vi "Measurement A.vi"(0 "Inputs":T1, 5 "Directory Path":path, 7 "First name":string, 9 "Last name":string, 11 "error in (no error)":errorcluster) -> (4 "Result":dbl, 6 "file or folder exists?":bool, 8 "Full name":string, 10 "dup path":path, 15 "error out":errorcluster)   [LabVIEW 2021]
uses:
  controls/Measurement Inputs.ctl
  controls/Offset value.ctl
  Reusables/controls/Username.ctl
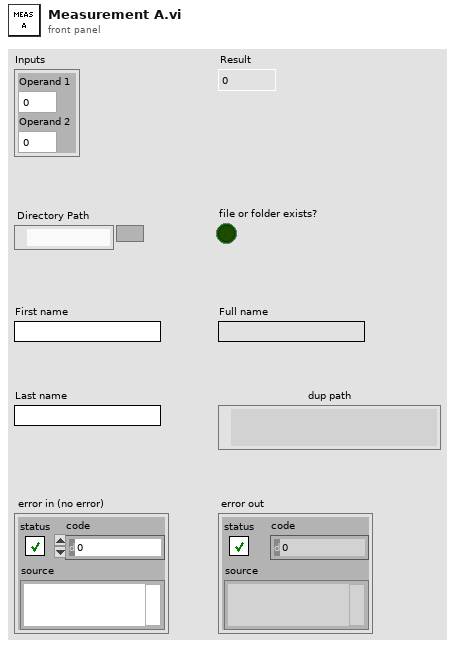
[diagram p1: front panel]
types:
  T1 = typedef "Measurement Inputs.ctl" = cluster{"Operand 1":dbl, "Operand 2":dbl}
  T2 = typedef "Username.ctl" = cluster{"First name":string, "Last name":string}
  T3 = typedef "Offset value.ctl" = cluster{"offset":dbl}
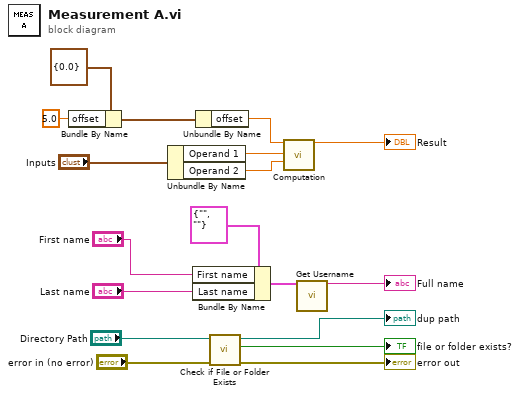
[diagram p0: block diagram]
diagram:
  n1 = Bundle By Name(cluster=T3 {"offset"=0.0}, "offset"=5.0) -> (w11:T3)
  n2 = Unbundle By Name("Inputs") -> ("Operand 1"=w17:dbl, "Operand 2"=w16:dbl)
  n3 = Bundle By Name(cluster=T2 {"First name"="", "Last name"=""} ("Name"), "First name"="First name", "Last name"="Last name") -> (w9:T2)
  n4 = Unbundle By Name(w11) -> ("offset"=w15:dbl)
  n5 = call <vilib>:"Check if File or Folder Exists.vi"("error in (no error)"="error in (no error)", "path"="Directory Path") -> ("error out"=→"error out":errorcluster, "file or folder exists?"=→"file or folder exists?":bool, "dup path"=→"dup path":path)  [unwired: 7 in]
  n6 = call "Computation.vi"("offset"=w15, "Operand 1"=w17, "Operand 2"=w16) -> ("Result"=→"Result":dbl)  [unwired: 12 in]
  n7 = call "Get Username.vi"("Name"=w9) -> ("Full name"=→"Full name":string)  [unwired: 14 in]
